vi "Set Report Font.vi"(0 "report in":refnum<class "ooWriter.lvclass">, 1 "text color (unchanged)":u32(colorbox)=16777216, 2 "font settings source":u16(ring) items=["VI Inputs", "Font Dialog Box"], 5 "text options":T2, 9 "font settings":T3={"Charset (-1)"=-1, "Weight (-1)"=-1, "Name"="", "Size"=" "}, 11 "error in (no error)":errorcluster) -> (4 "report out":refnum<class "ooWriter.lvclass">, 6 "font out":T1={"font name"="", "font size"=0.0, "bold"=0, "italic"=0, "underline"=0, "strike through"=0, "font color"=16777216} {"font size" format="%0.2f"; "strike through" items=["Unchanged", "Yes", "No"]; "underline" items=["Unchanged", "Yes", "No"]; "italic" items=["Unchanged", "Yes", "No"]; "bold" items=["Unchanged", "Yes", "No"]}, 15 "error out":errorcluster)   [LabVIEW 2009, in "ooWriter.lvclass"]
doc: "Sets the font properties of the report, including those in the headers and footers."
uses:
  ooWriter.lvclass
  <vilib>/Utility/NIReport.llb/font.ctl
  ooWriter.lvclass/ooWriter.ctl
  C:/Projets/LAVAG/OpenOfficeRGT/AODL/DLLs/AODL.dll
  <vilib>/Utility/NIReport.llb/NI_ReportGenerationCore.lvlib
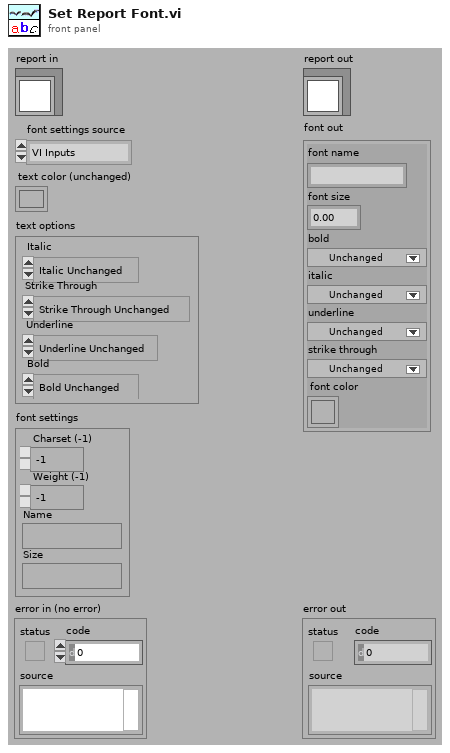
[diagram p1: front panel]
types:
  T1 = typedef "NI_ReportGenerationCore.lvlib/font.ctl" = cluster{"font name":string, "font size":dbl, "bold":u16, "italic":u16, "underline":u16, "strike through":u16, "font color":u32}
  T2 = cluster{"Italic":enum16{"Italic Unchanged", "Italic On", "Italic Off"}, "Strike Through":enum16{"Strike Through Unchanged", "Strike Through On", "Strike Through Off"}, "Underline":enum16{"Underline Unchanged", "Underline On", "Underline Off"}, "Bold":enum16{"Bold Unchanged", "Bold On", "Bold Off"}}
  T3 = cluster{"Charset (-1)":i16, "Weight (-1)":i16, "Name":string, "Size":string}
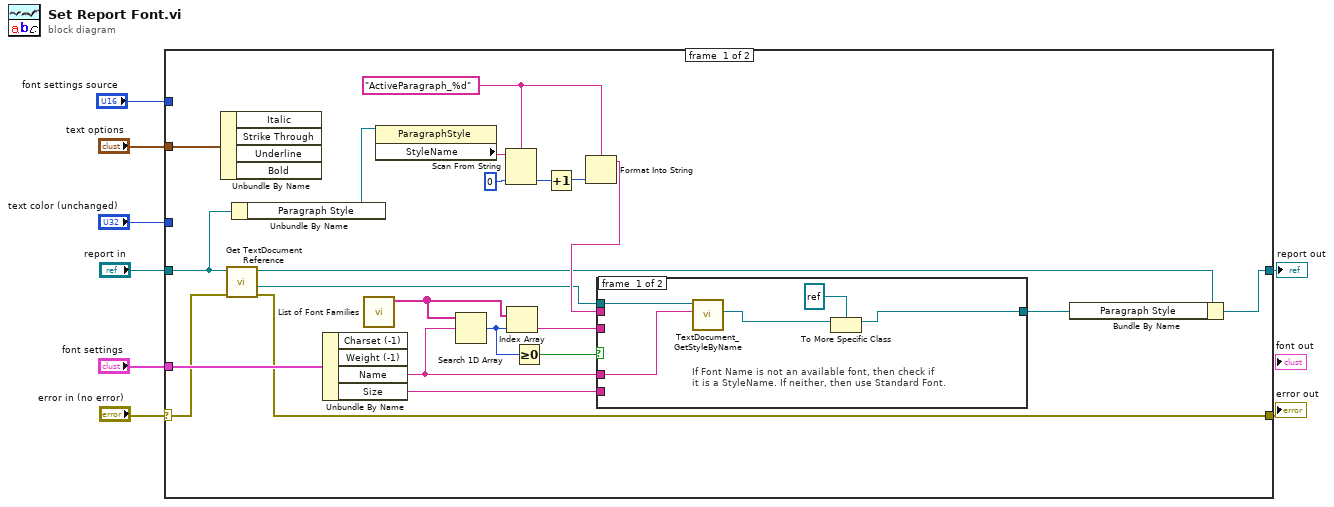
[diagram p0: block diagram]
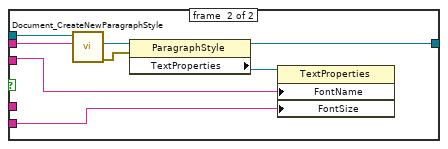
[diagram p2: hidden frame]
diagram:
  n1 = case shown="No Error" "error in (no error)" {
    selector: "error in (no error)" -> [w11 w44]
    tunnel: [w10 w44] -> w8
    tunnel: "report in" -> [w13 w45]
    tunnel: [w22 w45] -> w6
    tunnel: "font settings" -> [w29 _]
    tunnel: "text options" -> [w30 _]
    tunnel: "text color (unchanged)" -> [_ _]
    tunnel: "font settings source" -> [_ _]
    frame #0 {
      w23 = "ActiveParagraph_%d" ("styleName")
      n2 = Unbundle By Name(w30) -> ()  [unwired: 4 out]
      n3 = call-dynamic "Get TextDocument Reference.vi"("error in (no error)"=w11, "ooWriter in"=w13) -> ("error out"=w10:errorcluster, "Document"=w12:refnum<k24>, "ooWriter out"=w9:refnum<class "ooWriter.lvclass">)  [unwired: 7 in]
      n4 = Unbundle By Name(w13) -> ("Paragraph Style"=w28:refnum<k24>)
      n5 = Unbundle By Name(w29) -> ("Name"=w14:string, "Size"=w15:string)  [unwired: 2 out]
      n6 = call "List of Font Families.vi"() -> ("Available Fonts"=w21:string[])  [unwired: 11 in]
      n7 = property class="ParagraphStyle"(reference=w28) -> ("StyleName"=w27:string)  [unwired: 1 in, 2 out]
      n8 = Search 1D Array(1D array=w21, element=w14) -> (index of element=w20:i32)  [unwired: 1 in]
      n9 = Scan From String(format string=w23, input string=w27, default 1=0 ("default value 1")) -> (output 1=w25:i32)  [unwired: 2 in, 3 out]
      n10 = Index Array(array=w21, index=w20) -> (element=w16:string)
      n11 = Greater Or Equal To 0?(x=w20) -> (x >= 0?=w19:bool)
      n12 = Increment(x=w25) -> (x+1=w24:i32)
      n13 = Format Into String(format string=w23, w24) -> (resulting string=w17:string)  [unwired: 2 in, 1 out]
      n14 = case shown="False" w19 {
        tunnel: w12 -> [w35 w43]
        tunnel: [w32 w36] -> w18
        tunnel: w17 -> [_ w42]
        tunnel: w16 -> [_ w38]
        tunnel: w15 -> [_ w37]
        tunnel: w14 -> [w31 _]
        frame #0 {
          # "If Font Name is not an available font, then check if\nit is a StyleName. If neither, then use Standard Font."
          n15 = call "TextDocument_GetStyleByName.vi"("StyleName"=w31, "TextDocument in"=w35) -> ("Style"=w34:refnum<k24>)  [unwired: 7 in, 2 out]
          n16 = To More Specific Class(target class=refnum<k24> refnum, reference=w34) -> (specific class reference=w32:refnum<k24>)  [unwired: 1 in, 1 out]
        }
        frame #1 {
          n17 = call "Document_CreateNewParagraphStyle.vi"("styleName"=w42, "document"=w43) -> ("error out"=w40:errorcluster, "Paragraph Style"=w41:refnum<k24>)  [unwired: 7 in, 1 out]
          n18 = property class="ParagraphStyle"(reference=w41, error in=w40) -> (reference out=w36:refnum<k24>, "TextProperties"=w39:refnum<k24>)  [unwired: 1 out]
          n19 = property class="TextProperties"(reference=w39, "FontName"=w38, "FontSize"=w37) -> ()  [unwired: 1 in, 2 out]
        }
      }
      n20 = Bundle By Name(cluster=w9, "Paragraph Style"=w18) -> (w22:refnum<class "ooWriter.lvclass">)
    }
    frame #1 {
    }
  }
  "error out" <- w8
  "report out" <- w6
